vi "3D change Ant Pol.vi"(7 "error in (no error)":errorcluster caption="에러 입력(에러 없음)", 9 "Target Position (deg)":dbl, 10 "Instrument Manager 입력":refnum<class "Instrument Manager.lvclass">) -> (0 "error out":errorcluster caption="에러 출력", 1 "Current Position (degree)":dbl, 3 "Instrument Manager 출력":refnum<class "Instrument Manager.lvclass">)   [LabVIEW 2023, in "Instrument Manager.lvclass"]
uses:
  Instrument Manager.lvclass
  Instrument Manager.lvclass/Instrument Manager.ctl
  22dd40e7-a06b-45cc-aadf-926cb9933f1c.vi
  b9019dc1-b7cc-4ae5-aed8-9de0712302bb.vi
  Module/FCC FR2 3D Controller Module/Interface_3D Controller/Interface_3D Controller.lvclass
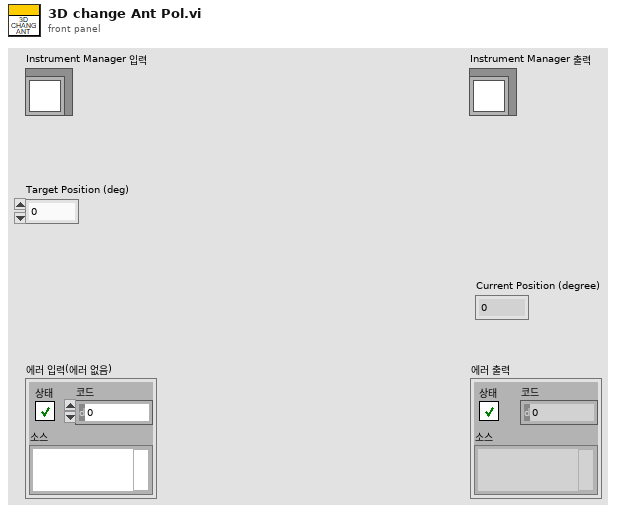
[diagram p1: front panel]
types:
  T1 = cluster{"Anritsu Call Box":refnum<class "Anritsu Call Box.lvclass">, "Spectrum Analyzer":refnum<class "Interface_Spectrum.lvclass">, "RF Switch Box":refnum<class "RF Filter Box.lvclass">, "Turn Table":refnum<class "Interface - Turn Table.lvclass">, "Mast":refnum<class "Interface - Mast.lvclass">, "3D Controller":refnum<class "Interface_3D Controller.lvclass">}
  T2 = typedef "FCC 3D Controller for BS.lvlib/TYPE Axis Parameter List.ctl" = cluster{"ACC/Deceleration(ms)":dbl, "Velocity (degree/sec)":dbl, "Target Position (degree)":dbl, "Current Position (degree)":dbl, "Limit Positive (degree)":dbl, "Limit Negative (degree)":dbl}
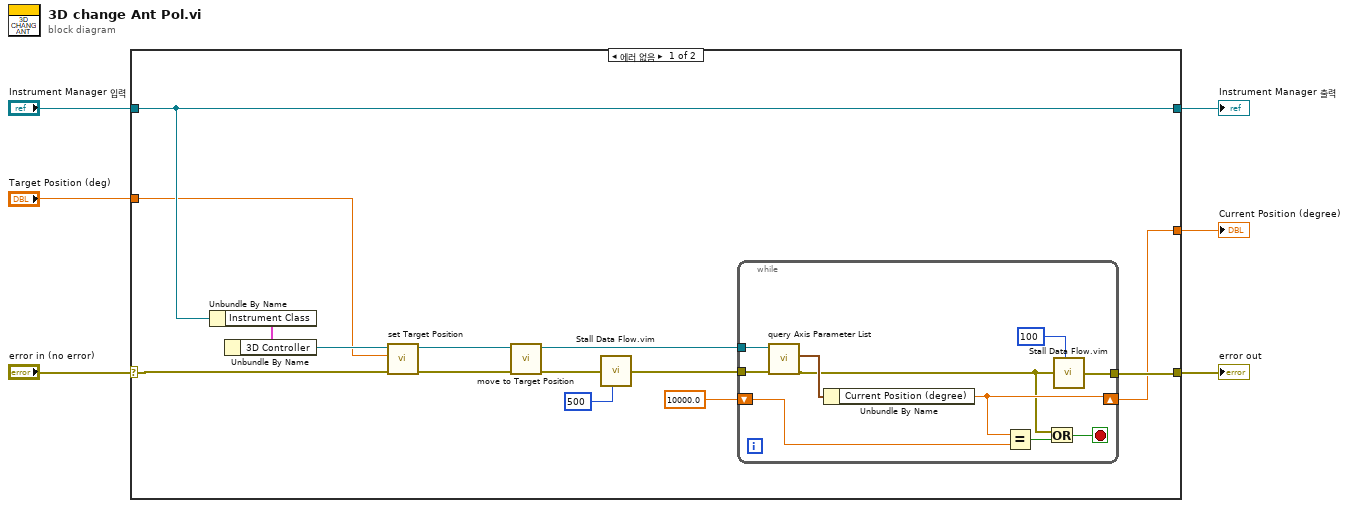
[diagram p0: block diagram]
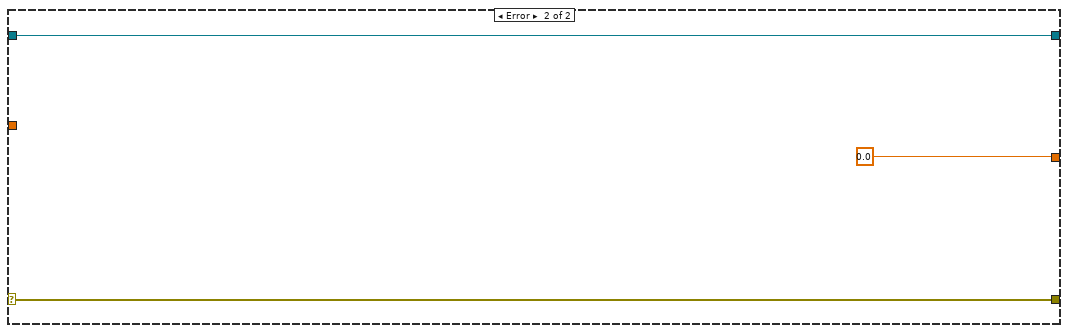
[diagram p2: hidden frame]
diagram:
  n1 = case shown="에러 없음" "error in (no error)" {
    selector: "error in (no error)" -> [w15 w33]
    tunnel: [w9 w33] -> w5
    tunnel: [w20 w32] -> w3
    tunnel: "Instrument Manager 입력" -> [w20 w32]
    tunnel: [w8 0.0 ("Current Position (degree)")] -> w2
    tunnel: "Target Position (deg)" -> [w7 _]
    frame No Error {
      n2 = Unbundle By Name(w20) -> ("Instrument Class"=w19:T1)
      n3 = Unbundle By Name(w19) -> ("3D Controller"=w18:refnum<class "Interface_3D Controller.lvclass">)
      n4 = call-dynamic "set Target Position.vi"("error in (no error)"=w15, "Target Position (deg)"=w7, "Interface_3D Controller in"=w18) -> ("error out"=w14:errorcluster, "Interface_3D Controller out"=w17:refnum<class "Interface_3D Controller.lvclass">)  [unwired: 7 in]
      n5 = call-dynamic "move to Target Position.vi"("error in (no error)"=w14, "Interface_3D Controller in"=w17) -> ("error out"=w13:errorcluster, "Interface_3D Controller out"=w16:refnum<class "Interface_3D Controller.lvclass">)  [unwired: 8 in]
      n6 = call "Stall Data Flow.vim"("value in"=w13, "milliseconds to wait"=u32 500) -> ("value out"=w11:errorcluster)  [unwired: 1 out]
      n7 = while {
        tunnel: w16 -> [w30]
        tunnel: w11 -> [w29]
        shift-right: [w26] -> w8
        shift-left: 10000.0 ("Current Position (degree)") -> [w27]
        tunnel: [w22] -> w9
        stop <- w24 stop-if-true
        n8 = call-dynamic "query Axis Parameter List.vi"("error in (no error)"=w29, "Interface_3D Controller in"=w30) -> ("error out"=w23:errorcluster, "Axis Parameter List"=w28:T2)  [unwired: 6 in, 2 out]
        n9 = Unbundle By Name(w28) -> ("Current Position (degree)"=w26:dbl)
        n10 = Equal?(x=w26, y=w27) -> (x = y?=w25:bool)
        n11 = Or(x=w23, y=w25) -> (x .or. y?=w24:bool)
        n12 = call "Stall Data Flow.vim"("value in"=w23, "milliseconds to wait"=u32 100) -> ("value out"=w22:errorcluster)  [unwired: 1 out]
      }
    }
    frame Error {
    }
  }
  "error out" <- w5
  "Instrument Manager 출력" <- w3
  "Current Position (degree)" <- w2
